vi "Dictionary to XY Graph.vi"(8 "error in (no error)":errorcluster, 11 "Results (Dictionary)":cluster{"key":string, "value":dbl[]}[](array[cluster])) -> (0 "error out":errorcluster, 2 "XY Graph":cluster{dbl[], dbl[]}[](array[cluster]), 3 "Results (Dictionary) out":cluster{"key":string, "value":dbl[]}[](array[cluster]))   [LabVIEW 2019, in "Instrument.Lockin.lvlib" / "Instrument UI.Lockin.lvclass"]
uses:
  Instrument UI.Lockin.lvclass
  Instrument.Lockin/Typedefs/Results Type--Enum.ctl
  Instrument.Lockin/Instrument.Lockin.lvclass
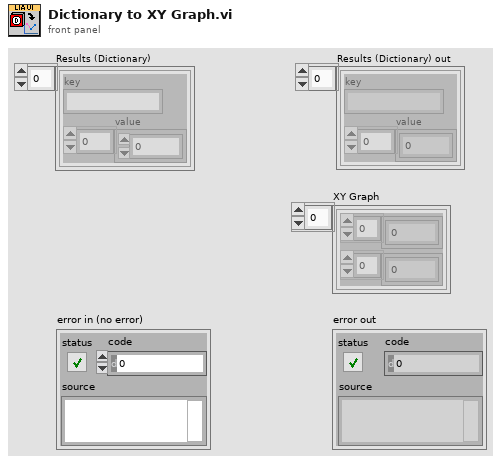
[diagram p1: front panel]
types:
  T1 = typedef "Instrument.Lockin.lvlib/Instrument.Lockin.lvclass/Results Type--Enum.ctl" = enum16{"X", "Y", "R", "Theta", "Mean"}
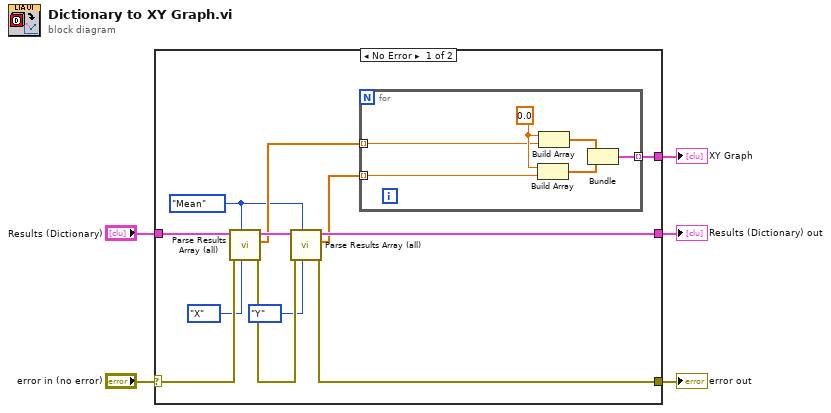
[diagram p0: block diagram]
diagram:
  n1 = case shown="No Error" "error in (no error)" {
    selector: "error in (no error)" -> [w15 w24]
    tunnel: "Results (Dictionary)" -> [w16 _]
    tunnel: [w12 w24] -> w3
    tunnel: [w17 _] -> w2
    tunnel: [w9 _] -> w1
    frame No Error {
      w6 = enum16{"Mean", "Sample"}."Mean" ("Processing")
      n2 = call "Parse Results Array (all).vi"("Type"=Results_Type--Enum."X", "Processing"=w6, "error in (no error)"=w15, "Results (Dictionary)"=w16) -> ("error out"=w13:errorcluster, "Data"=w8:dbl[], "Results (Dictionary)"=w14:cluster{"key":string, "value":dbl[]}[])  [unwired: 4 in, 1 out]
      n3 = call "Parse Results Array (all).vi"("Type"=Results_Type--Enum."Y", "Processing"=w6, "error in (no error)"=w13, "Results (Dictionary)"=w14) -> ("error out"=w12:errorcluster, "Data"=w7:dbl[], "Results (Dictionary)"=w9:cluster{"key":string, "value":dbl[]}[])  [unwired: 4 in, 1 out]
      n4 = for {
        tunnel: w8 -> [w19] mode=indexing
        tunnel: w7 -> [w18] mode=indexing
        tunnel: [w20] -> w17 mode=indexing
        w23 = 0.0
        n5 = Build Array(w23, w18) -> (w21:dbl[])
        n6 = Build Array(w23, w19) -> (w22:dbl[])
        n7 = Bundle(w22, w21) -> (w20:cluster{dbl[], dbl[]})  [unwired: 1 in]
      }
    }
    frame Error {
    }
  }
  "error out" <- w3
  "XY Graph" <- w2
  "Results (Dictionary) out" <- w1
